vi "_script_remove_all_csm_bookmarks.vi"(11 "Vi Path":path=path "D:/github/JKI-State-Machine-Plus/src/user.lib/_NEVSTOP/JKI State Machine++/JKISM++ No-Event Structure Template.vi") -> ()   [LabVIEW 2017]
uses:
  _csmHelper/API/Destroy.vi
  _csmHelper/API/Open Block Diagram.vi
  _csmHelper/API/Create From VI Reference.vi
  _csmHelper/CSM-Helper.lvclass
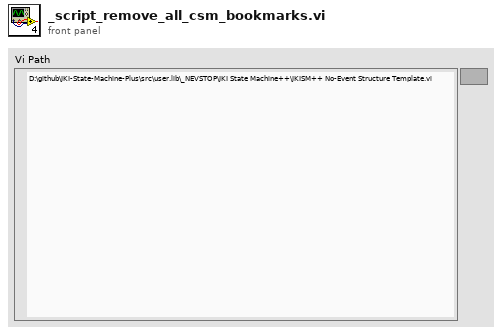
[diagram p1: front panel]
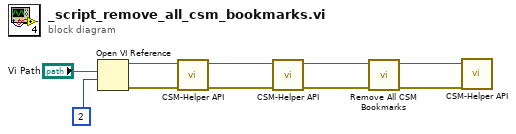
[diagram p0: block diagram]
diagram:
  n1 = Open VI Reference(vi path="Vi Path", options=2) -> (vi reference=w2:refnum<vi>, error out=w1:errorcluster)  [unwired: 4 in]
  n2 = call-poly "CSM-Helper API.vi"("error in (no error)"=w1, "VI"=w2) -> ("error out"=w8:errorcluster, "CSM-Helper.lvclass"=w7:refnum<class "CSM-Helper.lvclass">)  [unwired: 8 in]
  n3 = call-poly "CSM-Helper API.vi"("error in (no error)"=w8, "CSM-Helper in"=w7) -> ("error out"=w6:errorcluster, "CSM-Helper out"=w5:refnum<class "CSM-Helper.lvclass">)  [unwired: 8 in]
  n4 = call "Remove All CSM Bookmarks.vi"("error in (no error)"=w6, "CSM-Helper in"=w5) -> ("error out"=w4:errorcluster, "CSM-Helper out"=w3:refnum<class "CSM-Helper.lvclass">)  [unwired: 8 in]
  n5 = call-poly "CSM-Helper API.vi"("error in (no error)"=w4, "CSM-Helper in"=w3) -> ()  [unwired: 8 in, 2 out]
